vi "PLC Manual Write.vi"(9 "data":variant, 10 "station":string, 11 "URL":string) -> (0 "value":bool, 1 "autochange":bool, 2 "Value":u8[](array[numeric]), 3 "ok?":bool)   [LabVIEW 2012]
uses:
  Globals/Global.vi
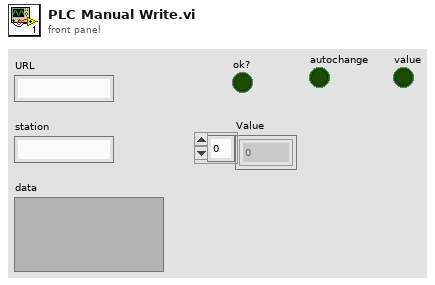
[diagram p1: front panel]
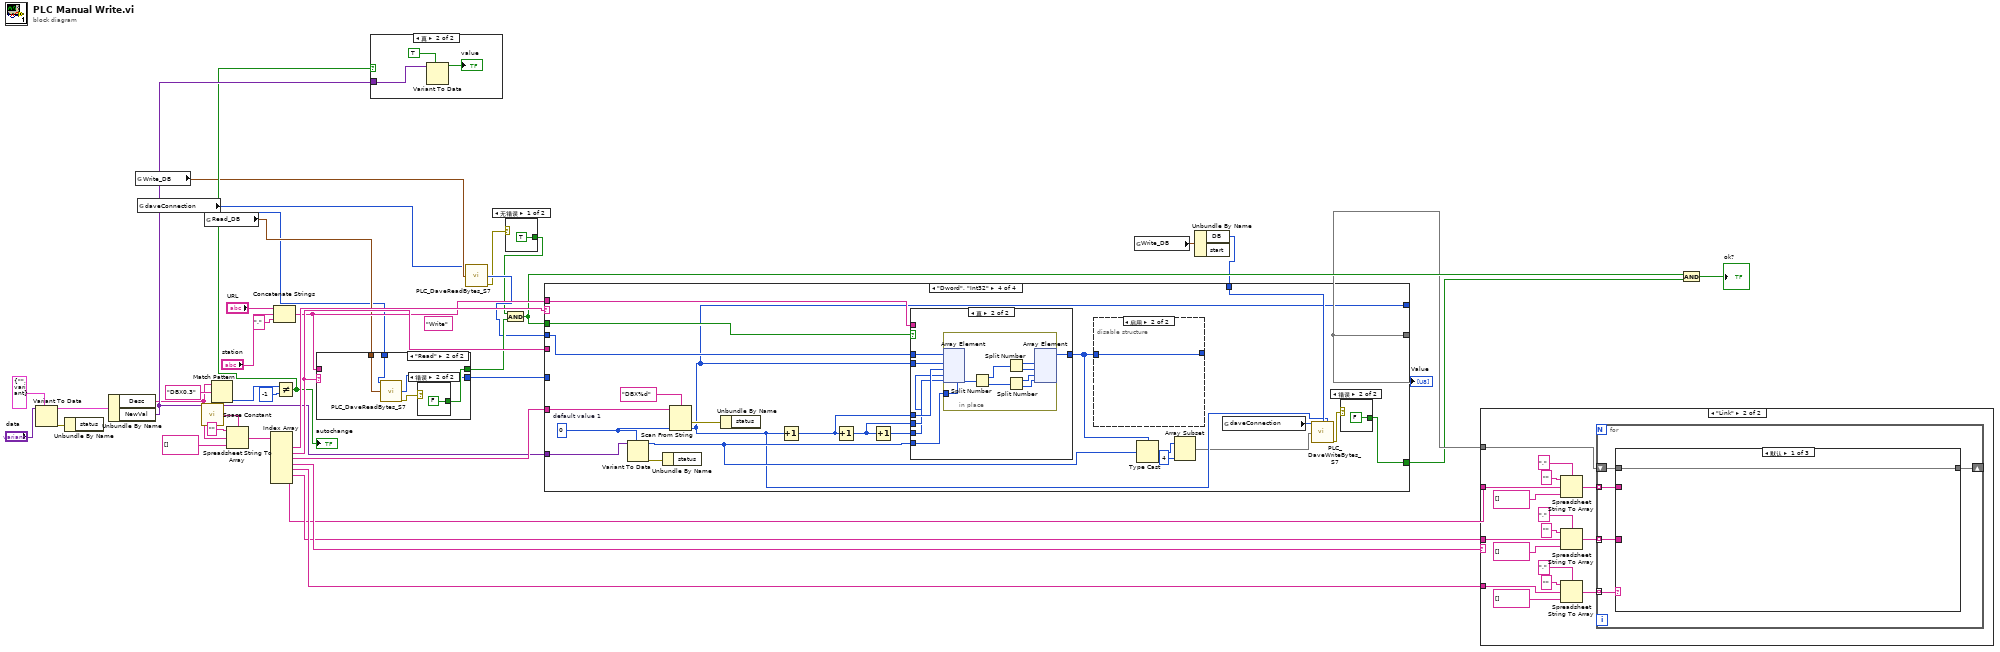
[diagram p0: block diagram]
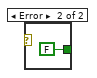
[diagram p2: hidden frame]
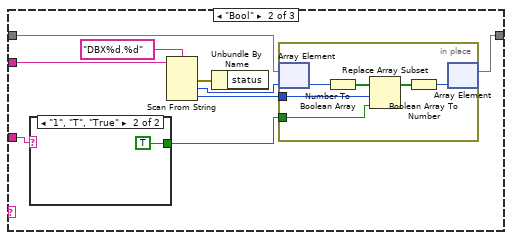
[diagram p5: hidden frame]
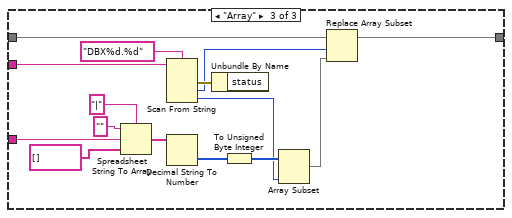
[diagram p7: hidden frame]
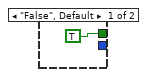
[diagram p8: hidden frame]
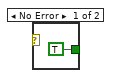
[diagram p9: hidden frame]
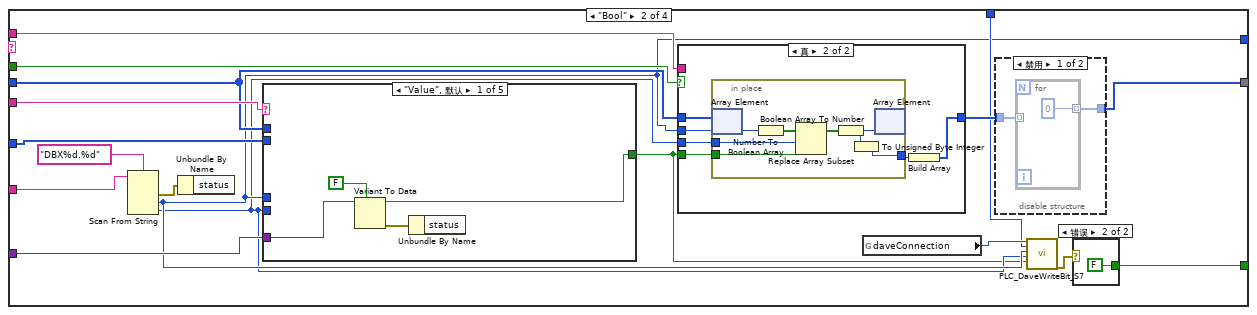
[diagram p11: hidden frame]
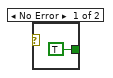
[diagram p12: hidden frame]
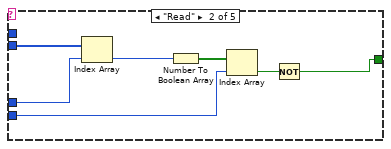
[diagram p14: hidden frame]
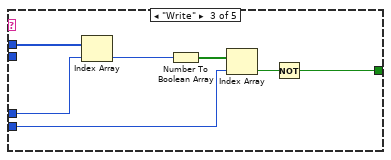
[diagram p15: hidden frame]
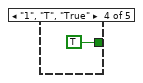
[diagram p16: hidden frame]
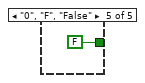
[diagram p17: hidden frame]
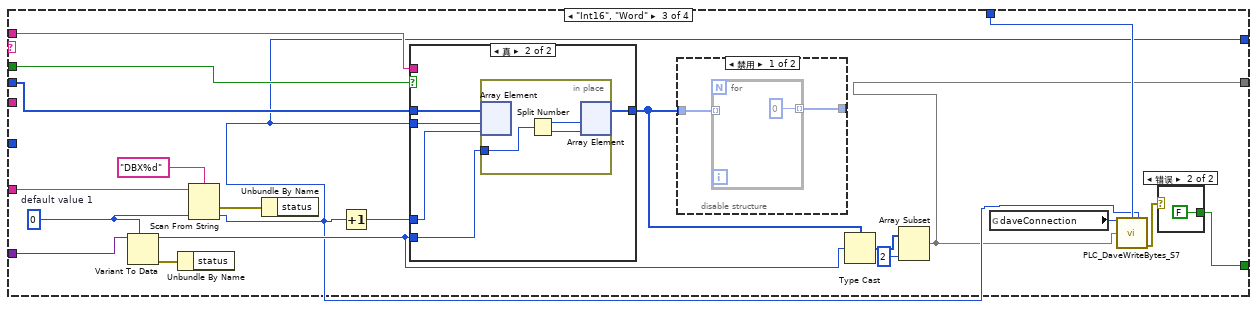
[diagram p19: hidden frame]
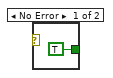
[diagram p20: hidden frame]
diagram:
  (unwired) "Write" ("Address")
  n1 = Variant To Data(type=cluster{"Desc":string, "NewVal":variant} {"Desc"="", "NewVal"=variant} ("output cluster"), Variant="data") -> (data=w38:cluster{"Desc":string, "NewVal":variant}, error out=w36:errorcluster)  [unwired: 1 in]
  n2 = Unbundle By Name(w36) -> ()  [unwired: 1 out]
  n3 = Unbundle By Name(w38) -> ("Desc"=w13:string, "NewVal"=w15:variant)
  n4 = global read "Global.vi" "Write_DB"() -> (w9:cluster{"DB":i32, "start":i32, "len":i32})
  n5 = global read "Global.vi" "daveConnection"() -> (w6:i64)
  n6 = call <vilib>:"Space Constant.vi"() -> ("String"=w21:string)
  n7 = global read "Global.vi" "Read_DB"() -> (w7:cluster{"DB":i32, "start":i32, "len":i32})
  n8 = Match Pattern(string=w13, regular expression="DBX0.3" ("y")) -> (offset past match=w12:i32)  [unwired: 1 in, 3 out]
  n9 = Spreadsheet String To Array(delimiter (Tab)=w21, format string="", spreadsheet string=w13, array type (2D Dbl)=string[] []) -> (array=w30:string[])
  n10 = Index Array(array=w30) -> (element #1=w29:string, element #2=w27:string, element #3=w28:string, element #4=w20:string, element #5=w19:string, element #6=w18:string, element #7=w16:string)  [unwired: 7 in]
  n11 = Concatenate Strings("URL", "station", "." ("string")) -> (w26:string)
  n12 = Not Equal?(x=w12, y=-1) -> (x != y?=w10:bool)
  "autochange" <- w10
  n13 = case shown="\"Read\"" w27 {
    tunnel: w26 -> [_ _]
    tunnel: [TRUE ("ok?") w42] -> w25
    tunnel: [_ w41] -> w23
    tunnel: w7 -> [_ w45]
    tunnel: w6 -> [_ w44]
    frame "False", Default {
    }
    frame "Read" {
      n14 = call "PLC_DaveReadBytes_S7.vi"("daveConnection in"=w44, "地址"=w45) -> ("read Buffer"=w41:u8[], "error out"=w43:errorcluster)  [unwired: 10 in, 2 out]
      n15 = case shown="错误" w43 {
        tunnel: [TRUE FALSE] -> w42
        frame No Error {
        }
        frame Error {
        }
      }
    }
  }
  n16 = case shown="真" w10 {
    tunnel: w15 -> [_ w50]
    frame False {
    }
    frame True {
      n17 = Variant To Data(type=TRUE, Variant=w50) -> (data=→"value":bool)  [unwired: 1 in, 1 out]
    }
  }
  n18 = call "PLC_DaveReadBytes_S7.vi"("daveConnection in"=w6, "地址"=w9) -> ("read Buffer"=w8:u8[], "error out"=w5:errorcluster)  [unwired: 10 in, 2 out]
  n19 = case shown="无错误" w5 {
    tunnel: [TRUE FALSE] -> w4
    frame No Error {
    }
    frame Error {
    }
  }
  n20 = And(x=w4, y=w25) -> (x .and. y?=w24:bool)
  n21 = global read "Global.vi" "Write_DB"() -> (w3:cluster{"DB":i32, "start":i32, "len":i32})
  n22 = Unbundle By Name(w3) -> ("DB"=w2:i32)  [unwired: 1 out]
  n23 = case shown="\"Dword\", \"Int32\"" w29 {
    tunnel: w15 -> [_ w71 w130 w166]
    tunnel: w8 -> [w53 w63 w124 w160]
    tunnel: w26 -> [_ w70 w129 w165]
    tunnel: [w53 w61 w112 _] -> w17
    tunnel: w24 -> [_ w69 w128 w164]
    tunnel: w28 -> [_ w64 w125 w161]
    tunnel: w27 -> [_ w68 _ _]
    tunnel: w23 -> [_ w67 _ _]
    tunnel: [_ w58 w113 w147] -> _
    tunnel: w2 -> [_ w59 w114 w148]
    tunnel: [_ w54 w111 w145] -> w1
    frame "False", Default {
    }
    frame "Bool" {
      n24 = Scan From String(format string="DBX%d.%d" ("regular expression"), input string=w64) -> (error out=w66:errorcluster, output 1=w58:i32, output 2=w57:i32)  [unwired: 4 in, 2 out]
      n25 = Unbundle By Name(w66) -> ()  [unwired: 1 out]
      n26 = case shown="\"Value\", 默认" w68 {
        tunnel: [w78 w82 w89 TRUE ("status") FALSE ("status")] -> w56
        tunnel: w71 -> [w80 _ _ _ _]
        tunnel: w67 -> [_ w88 _ _ _]
        tunnel: w58 -> [_ w85 w93 _ _]
        tunnel: w57 -> [_ w84 w92 _ _]
        tunnel: w63 -> [_ _ w91 _ _]
        frame "Value", Default {
          n27 = Variant To Data(type=FALSE ("status"), Variant=w80) -> (data=w78:bool, error out=w81:errorcluster)  [unwired: 1 in]
          n28 = Unbundle By Name(w81) -> ()  [unwired: 1 out]
        }
        frame "Read" {
          n29 = Index Array(array=w88, index=w85) -> (element=w86:u8)
          n30 = Number To Boolean Array(number=w86) -> (Boolean array=w87:bool[])
          n31 = Index Array(array=w87, index=w84) -> (element=w83:bool)
          n32 = Not(x=w83) -> (.not. x?=w82:bool)
        }
        frame "Write" {
          n33 = Index Array(array=w91, index=w93) -> (element=w94:u8)
          n34 = Number To Boolean Array(number=w94) -> (Boolean array=w95:bool[])
          n35 = Index Array(array=w95, index=w92) -> (element=w90:bool)
          n36 = Not(x=w90) -> (.not. x?=w89:bool)
        }
        frame "1", "T", "True" {
        }
        frame "0", "F", "False" {
        }
      }
      n37 = case shown="真" w69 {
        tunnel: w70 -> [_ _]
        tunnel: w63 -> [_ w103]
        tunnel: w56 -> [_ w102]
        tunnel: [_ w98] -> w62
        tunnel: w58 -> [_ w101]
        tunnel: w57 -> [_ w100]
        frame False {
        }
        frame True {
          n38 = in-place {
            in-place-border: w100 -> [w108]
            in-place-border: w102 -> [w107]
            in-place-border: [w104] -> w99
            n39 = in-place-array #1(w103, w101) -> (w110:u8)
            n40 = Number To Boolean Array(number=w110) -> (Boolean array=w109:bool[])
            n41 = Replace Array Subset(array=w109, new element=w107, index=w108) -> (w106:bool[])
            n42 = Boolean Array To Number(Boolean array=w106) -> (number=w105:u32)
            n43 = To Unsigned Byte Integer(number=w105) -> (unsigned 8bit integer=w104:u8)
            n44 = in-place-array #1(w105) -> ()  [unwired: 2 out]
          }
          n45 = Build Array(w99) -> (w98:u8[])
        }
      }
      n46 = global read "Global.vi" "daveConnection"() -> (w60:i64)
      n47 = disable-structure shown="禁用" {
        disable-tunnel: w62 -> [w75 w77]
        disable-tunnel: [w74 w77] -> w61
        frame Disabled {
          n48 = for {
            tunnel: w75 -> [_] mode=indexing
            tunnel: [u8 0 ("数值")] -> w74 mode=indexing
          }
        }
        frame Enabled {
        }
      }
      n49 = call "PLC_DaveWriteBit_S7.vi"("daveConnection IN"=w60, "DB"=w59, "byte"=w58, "bit"=w57, "value"=w56) -> ("error out"=w55:errorcluster)  [unwired: 12 in, 2 out]
      n50 = case shown="错误" w55 {
        tunnel: [TRUE FALSE] -> w54
        frame No Error {
        }
        frame Error {
        }
      }
    }
    frame "Int16", "Word" {
      w122 = i16 0  # default value 1
      n51 = Variant To Data(type=w122, Variant=w130) -> (data=w120:i16, error out=w123:errorcluster)  [unwired: 1 in]
      n52 = Unbundle By Name(w123) -> ()  [unwired: 1 out]
      n53 = Scan From String(format string="DBX%d" ("regular expression"), input string=w125, default 1=w122) -> (error out=w127:errorcluster, output 1=w113:i16)  [unwired: 2 in, 2 out]
      n54 = Unbundle By Name(w127) -> ()  [unwired: 1 out]
      n55 = Increment(x=w113) -> (x+1=w121:i16)
      n56 = case shown="真" w128 {
        tunnel: w129 -> [_ _]
        tunnel: w124 -> [_ w141]
        tunnel: w120 -> [_ w138]
        tunnel: [_ w140] -> w119
        tunnel: w113 -> [_ w139]
        tunnel: w121 -> [_ w137]
        frame False {
        }
        frame True {
          n57 = in-place {
            in-place-border: w138 -> [w144]
            n58 = in-place-array #2(w141, w139, w137) -> ()  [unwired: 2 out]
            n59 = Split Number(x=w144) -> (hi(x)=w143:u8, lo(x)=w142:u8)
            n60 = in-place-array #2(w143, w142) -> (w140:u8[])  [unwired: 2 out]
          }
        }
      }
      n61 = disable-structure shown="禁用" {
        disable-tunnel: w119 -> [w134 w136]
        disable-tunnel: [w133 w136] -> _
        frame Disabled {
          n62 = for {
            tunnel: w134 -> [_] mode=indexing
            tunnel: [u8 0 ("数值")] -> w133 mode=indexing
          }
        }
        frame Enabled {
        }
      }
      n63 = Type Cast(type=w119, x=w120) -> (*(type *) &x=w118:u8[])
      n64 = Array Subset(array=w118, length=2 ("长度")) -> (w112:u8[])  [unwired: 1 in]
      n65 = global read "Global.vi" "daveConnection"() -> (w115:i64)
      n66 = call "PLC_DaveWriteBytes_S7.vi"("daveConnectionIN"=w115, "DB"=w114, "start"=w113, "Buffer"=w112) -> ("error out"=w116:errorcluster)  [unwired: 9 in, 2 out]
      n67 = case shown="错误" w116 {
        tunnel: [TRUE FALSE] -> w111
        frame No Error {
        }
        frame Error {
        }
      }
    }
    frame "Dword", "Int32" {
      w158 = 0  # default value 1
      n68 = Variant To Data(type=w158, Variant=w166) -> (data=w152:i32, error out=w159:errorcluster)  [unwired: 1 in]
      n69 = Unbundle By Name(w159) -> ()  [unwired: 1 out]
      n70 = Scan From String(format string="DBX%d" ("regular expression"), input string=w161, default 1=w158) -> (error out=w163:errorcluster, output 1=w147:i32)  [unwired: 2 in, 2 out]
      n71 = Unbundle By Name(w163) -> ()  [unwired: 1 out]
      n72 = Increment(x=w147) -> (x+1=w157:i32)
      n73 = Increment(x=w157) -> (x+1=w156:i32)
      n74 = Increment(x=w156) -> (x+1=w155:i32)
      n75 = case shown="真" w164 {
        tunnel: w165 -> [_ _]
        tunnel: w160 -> [_ w179]
        tunnel: w152 -> [_ w176]
        tunnel: [_ w178] -> w151
        tunnel: w147 -> [_ w177]
        tunnel: w157 -> [_ w175]
        tunnel: w156 -> [_ w174]
        tunnel: w155 -> [_ w173]
        frame False {
        }
        frame True {
          n76 = in-place {
            in-place-border: w176 -> [w186]
            n77 = in-place-array #3(w179, w177, w175, w174, w173) -> ()  [unwired: 4 out]
            n78 = Split Number(x=w186) -> (hi(x)=w185:u16, lo(x)=w184:u16)
            n79 = Split Number(x=w185) -> (hi(x)=w183:u8, lo(x)=w182:u8)
            n80 = Split Number(x=w184) -> (hi(x)=w181:u8, lo(x)=w180:u8)
            n81 = in-place-array #3(w183, w182, w181, w180) -> (w178:u8[])  [unwired: 4 out]
          }
        }
      }
      n82 = disable-structure shown="启用" {
        disable-tunnel: w151 -> [w170 w172]
        disable-tunnel: [w169 w172] -> _
        frame Disabled {
          n83 = for {
            tunnel: w170 -> [_] mode=indexing
            tunnel: [u8 0 ("数值")] -> w169 mode=indexing
          }
        }
        frame Enabled {
        }
      }
      n84 = Type Cast(type=w151, x=w152) -> (*(type *) &x=w154:u8[])
      n85 = Array Subset(array=w154, length=4 ("长度")) -> (w146:u8[])  [unwired: 1 in]
      n86 = global read "Global.vi" "daveConnection"() -> (w149:i64)
      n87 = call "PLC_DaveWriteBytes_S7.vi"("daveConnectionIN"=w149, "DB"=w148, "start"=w147, "Buffer"=w146) -> ("error out"=w150:errorcluster)  [unwired: 9 in, 2 out]
      n88 = case shown="错误" w150 {
        tunnel: [TRUE FALSE] -> w145
        frame No Error {
        }
        frame Error {
        }
      }
    }
  }
  "Value" <- w17
  n89 = case shown="\"Link\"" w20 {
    tunnel: w19 -> [_ w200]
    tunnel: w18 -> [_ w195]
    tunnel: w17 -> [_ w192]
    tunnel: w16 -> [_ w188]
    frame "False", Default {
    }
    frame "Link" {
      n90 = Spreadsheet String To Array(delimiter (Tab)=",", format string="", spreadsheet string=w188, array type (2D Dbl)=string[] []) -> (array=w187:string[])
      n91 = Spreadsheet String To Array(delimiter (Tab)=",", format string="", spreadsheet string=w195, array type (2D Dbl)=string[] []) -> (array=w193:string[])
      n92 = Spreadsheet String To Array(delimiter (Tab)=",", format string="", spreadsheet string=w200, array type (2D Dbl)=string[] []) -> (array=w194:string[])
      n93 = for {
        tunnel: w194 -> [w205] mode=indexing
        tunnel: w193 -> [w203] mode=indexing
        shift-right: [w206] -> _
        shift-left: w192 -> [w207]
        tunnel: w187 -> [w204] mode=indexing
        n94 = case shown="默认" w205 {
          tunnel: w207 -> [w208 w214 w230]
          tunnel: [w208 w213 w225] -> w206
          tunnel: w204 -> [_ w215 w237]
          tunnel: w203 -> [_ w210 w233]
          frame Default {
          }
          frame "Bool" {
            n95 = case shown="\"1\", \"T\", \"True\"" w210 {
              tunnel: [_ TRUE ("status")] -> w209
              frame "False", Default {
              }
              frame "1", "T", "True" {
              }
            }
            n96 = Scan From String(format string="DBX%d.%d" ("regular expression"), input string=w215) -> (error out=w217:errorcluster, output 1=w212:i32, output 2=w211:i32)  [unwired: 4 in, 2 out]
            n97 = Unbundle By Name(w217) -> ()  [unwired: 1 out]
            n98 = in-place {
              in-place-border: w211 -> [w222]
              in-place-border: w209 -> [w221]
              n99 = in-place-array #4(w214, w212) -> (w224:u8)
              n100 = Number To Boolean Array(number=w224) -> (Boolean array=w223:bool[])
              n101 = Replace Array Subset(array=w223, new element=w221, index=w222) -> (w220:bool[])
              n102 = Boolean Array To Number(Boolean array=w220) -> (number=w219:u32)
              n103 = in-place-array #4(w219) -> (w213:u8[])  [unwired: 1 out]
            }
          }
          frame "Array" {
            n104 = Spreadsheet String To Array(delimiter (Tab)="|", format string="", spreadsheet string=w233, array type (2D Dbl)=string[] []) -> (array=w232:string[])
            n105 = Scan From String(format string="DBX%d.%d" ("regular expression"), input string=w237) -> (error out=w239:errorcluster, output 1=w228:i32, output 2=w227:i32)  [unwired: 4 in, 2 out]
            n106 = Decimal String To Number(string=w232) -> (number=w231:i32[])  [unwired: 2 in, 1 out]
            n107 = Unbundle By Name(w239) -> ()  [unwired: 1 out]
            n108 = To Unsigned Byte Integer(number=w231) -> (unsigned 8bit integer=w229:u8[])
            n109 = Array Subset(array=w229, length=w227) -> (w226:u8[])  [unwired: 1 in]
            n110 = Replace Array Subset(array=w230, new element=w226, index=w228) -> (w225:u8[])
          }
        }
      }
    }
  }
  n111 = And(x=w24, y=w1) -> (x .and. y?=→"ok?":bool)
